vi "onTestExecution.vi"(6 "timeout (2000 ms)":i32=2000, 7 "Name":string, 8 "error in (no error)":errorcluster, 11 "Test Runner.Project in":refnum<class "Test Runner.Project.lvclass">) -> (0 "error out":errorcluster, 3 "Test Runner.Project out":refnum<class "Test Runner.Project.lvclass">)   [LabVIEW 2020, in "Caraya.lvlib" / "Test Runner.Project.lvclass"]
uses:
  Test Runner.Project.lvclass
  C:/projects/caraya/src/classes/Test Runner/Test Runner.lvclass
  Test Runner/Test Runner.lvclass
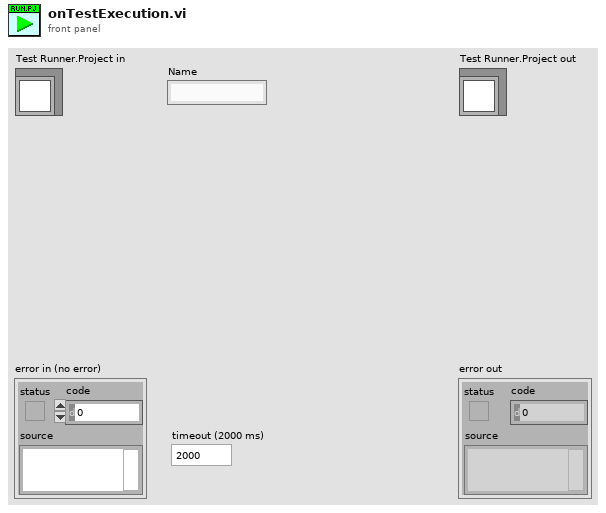
[diagram p1: front panel]
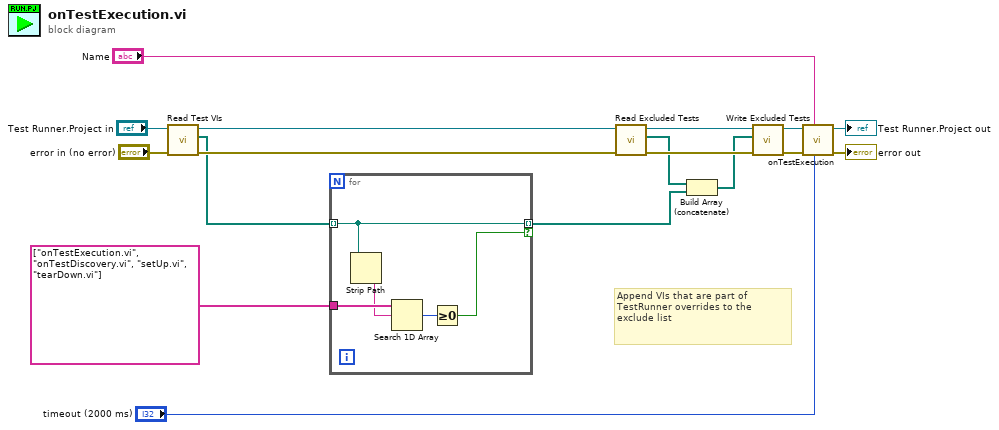
[diagram p0: block diagram]
diagram:
  # "Append VIs that are part of TestRunner overrides to the exclude list"
  n1 = call "Read Test VIs.vi"("error in (no error)"="error in (no error)", "Test Runner in"="Test Runner.Project in") -> ("error out"=w7:errorcluster, "Test VIs"=w4:path[], "Test Runner out"=w9:refnum<class "Test Runner.Project.lvclass">)  [unwired: 7 in]
  n2 = for {
    tunnel: w4 -> [w22] mode=indexing
    tunnel: [w22] -> w3 mode=indexing if=w18
    tunnel: string[] ["onTestExecution.vi", "onTestDiscovery.vi", "setUp.vi", "tearDown.vi"] -> [w21]
    n3 = Strip Path(path=w22) -> (name=w20:string)  [unwired: 1 out]
    n4 = Search 1D Array(1D array=w21, element=w20) -> (index of element=w19:i32)  [unwired: 1 in]
    n5 = Greater Or Equal To 0?(x=w19) -> (x >= 0?=w18:bool)
  }
  n6 = call "Read Excluded Tests.vi"("error in (no error)"=w7, "Test Runner in"=w9) -> ("error out"=w14:errorcluster, "Excluded Tests"=w6:path[], "Test Runner out"=w12:refnum<class "Test Runner.Project.lvclass">)  [unwired: 7 in]
  n7 = Build Array (concatenate)(w6, w3) -> (w5:path[])
  n8 = call "Write Excluded Tests.vi"("error in (no error)"=w14, "Excluded Tests"=w5, "Test Runner in"=w12) -> ("error out"=w13:errorcluster, "Test Runner out"=w11:refnum<class "Test Runner.Project.lvclass">)  [unwired: 7 in]
  n9 = call-parent "onTestExecution.vi"("timeout (2000 ms)"="timeout (2000 ms)", "Name"="Name", "error in (no error)"=w13, "Test Runner in"=w11) -> ("error out"=→"error out":errorcluster, "Test Runner out"=→"Test Runner.Project out":refnum<class "Test Runner.Project.lvclass">)  [unwired: 6 in]
